vi "Test Time Entry Month Files.vi"(8 "error in (no error)":errorcluster, 10 "Work Folder":path, 11 "Test Data Folder":path) -> (0 "error out":errorcluster, 2 "Report":string, 3 "Passed":bool)   [LabVIEW 2024]
doc: "Saves two entries with Time Entry Store-INI: one that starts on 30 Sep 2025 22:30 UTC (already 1 October in Central European time, and saved while today is in October) and one that runs from 31 Oct 23:30 UTC into November. The month file is chosen by the UTC Start Time, so the first must land in 2025-09.ini only and the second in 2025-10.ini only.\n\nInputs: Test Data Folder holds the source copies (Samples, v1); each run works in a new case folder under Work Folder. Passed is TRUE when every check passed and no error occurred; Report lists every check.\n\nGenerated by: Claude"
uses:
  Storage/Project Store-INI/Project Store-INI.lvclass
  Storage/Time Entry Store-INI/Time Entry Store-INI.lvclass
  Utilities/Time Management/Time Management.lvlib
  Storage/Time Entry Store/Time Entry Store.lvclass
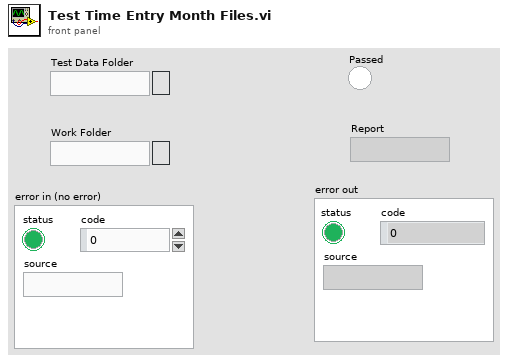
[diagram p1: front panel]
types:
  T1 = cluster{"c6018":string, "c6019":string, "c6020":string, "Timestamp":timestamp, "Timestamp":timestamp, "c6021":string}
  T2 = typedef "Time Entry.ctl" = cluster{"ID":string, "Project ID":string, "Task ID":string, "Start Time":timestamp, "End Time":timestamp, "Description":string}
  T3 = cluster{"c6030":string, "c6031":string, "c6032":string, "Timestamp":timestamp, "Timestamp":timestamp, "c6033":string}
  T4 = typedef "Time Entry List.ctl" = T2[]
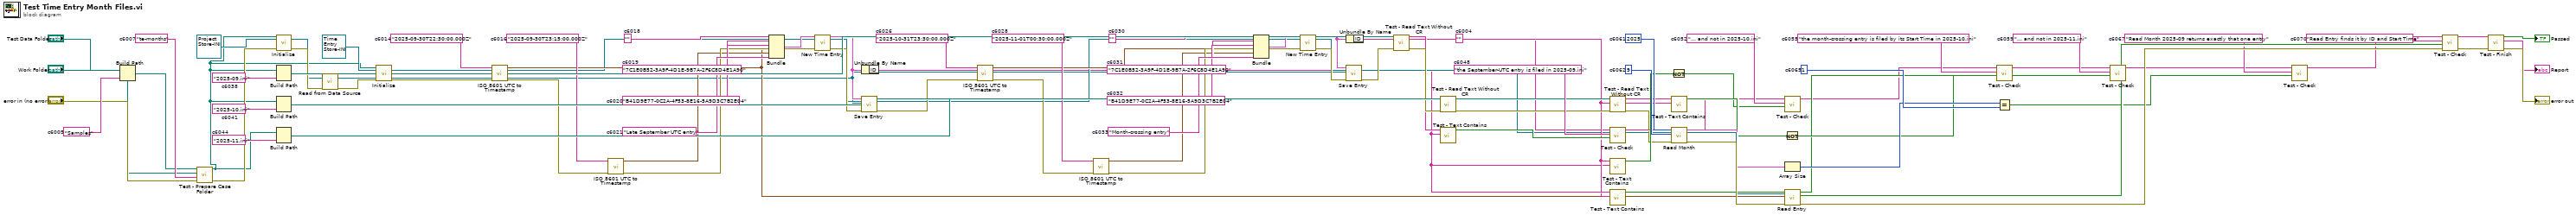
[diagram p0: block diagram]
diagram:
  w90 = "Read Entry finds it by ID and Start Time"  # c6070
  w86 = "Read Month 2025-09 returns exactly that one entry"  # c6067
  w84 = 1  # c6065
  w79 = 9  # c6062
  w78 = 2025  # c6061
  w76 = "... and not in 2025-11.ini"  # c6059
  w72 = "the month-crossing entry is filed by its Start Time in 2025-10.ini"  # c6055
  w69 = "... and not in 2025-10.ini"  # c6052
  w65 = "the September-UTC entry is filed in 2025-09.ini"  # c6048
  w60 = "2025-11.ini"  # c6044
  w56 = "2025-10.ini"  # c6041
  w52 = "2025-09.ini"  # c6038
  w44 = "Month-crossing entry"  # c6033
  w43 = "B41D9E77-0C2A-4F53-8E16-5A9D3C7B2E04"  # c6032
  w42 = "7C1E0B52-3A9F-4D1E-9B7A-2F6C8D4E1A90"  # c6031
  w41 = ""  # c6030
  w38 = "2025-11-01T00:30:00.000Z"  # c6028
  w35 = "2025-10-31T23:30:00.000Z"  # c6026
  w27 = "Late September UTC entry"  # c6021
  w26 = "B41D9E77-0C2A-4F53-8E16-5A9D3C7B2E04"  # c6020
  w25 = "7C1E0B52-3A9F-4D1E-9B7A-2F6C8D4E1A90"  # c6019
  w24 = ""  # c6018
  w21 = "2025-09-30T23:15:00.000Z"  # c6016
  w18 = "2025-09-30T22:30:00.000Z"  # c6014
  w7 = "te-months"  # c6007
  w5 = "Samples"  # c6005
  w4 = ""  # c6004
  n1 = Build Path(base path="Test Data Folder", name or relative path=w5) -> (appended path=w6:path)
  n2 = call "Test - Prepare Case Folder.vi"("error in (no error)"="error in (no error)", "Case Name"=w7, "Work Folder"="Work Folder", "Source Folder"=w6) -> ("error out"=w9:errorcluster, "Case Folder"=w8:path)  [unwired: 6 in]
  n3 = call-dynamic "Initialize.vi"("Project Store in"=refnum<class "Project Store-INI.lvclass"> refnum ("Project Store-INI"), "error in (no error)"=w9, "Data Folder"=w8) -> ("error out"=w12:errorcluster, "Project Store out"=w11:refnum<class "Project Store-INI.lvclass">)  [unwired: 7 in]
  n4 = Build Path(base path=w8, name or relative path=w52) -> (appended path=w53:path)
  n5 = Build Path(base path=w8, name or relative path=w56) -> (appended path=w57:path)
  n6 = Build Path(base path=w8, name or relative path=w60) -> (appended path=w61:path)
  n7 = call-dynamic "Read from Data Source.vi"("Project Store in"=w11, "error in (no error)"=w12) -> ("error out"=w14:errorcluster, "Project Store out"=w13:refnum<class "Project Store-INI.lvclass">)  [unwired: 8 in]
  n8 = call-dynamic "Initialize.vi"("Time Entry Store in"=refnum<class "Time Entry Store-INI.lvclass"> refnum ("Time Entry Store-INI"), "error in (no error)"=w14, "Data Folder"=w8) -> ("error out"=w17:errorcluster, "Time Entry Store out"=w16:refnum<class "Time Entry Store-INI.lvclass">)  [unwired: 7 in]
  n9 = call "ISO 8601 UTC to Timestamp.vi"("error in (no error)"=w17, "ISO 8601 UTC"=w18) -> ("error out"=w20:errorcluster, "Timestamp"=w19:timestamp)  [unwired: 8 in]
  n10 = call "ISO 8601 UTC to Timestamp.vi"("error in (no error)"=w20, "ISO 8601 UTC"=w21) -> ("error out"=w23:errorcluster, "Timestamp"=w22:timestamp)  [unwired: 8 in]
  n11 = Bundle("c6018"=w24, "c6019"=w25, "c6020"=w26, "Timestamp"=w19, "Timestamp"=w22, "c6021"=w27) -> (w28:T1)  [unwired: 1 in]
  n12 = call "New Time Entry.vi"("Time Entry Store in"=w16, "error in (no error)"=w23, "Time Entry"=w28) -> ("error out"=w31:errorcluster, "New Time Entry"=w29:T2, "Time Entry Store out"=w30:refnum<class "Time Entry Store-INI.lvclass">)  [unwired: 6 in]
  n13 = Unbundle By Name(w29) -> ("ID"=w32:string)
  n14 = call-dynamic "Save Entry.vi"("Time Entry Store in"=w30, "error in (no error)"=w31, "Project Store"=w13, "Time Entry"=w29) -> ("error out"=w34:errorcluster, "Time Entry Store out"=w33:refnum<class "Time Entry Store-INI.lvclass">)  [unwired: 6 in]
  n15 = call "ISO 8601 UTC to Timestamp.vi"("error in (no error)"=w34, "ISO 8601 UTC"=w35) -> ("error out"=w37:errorcluster, "Timestamp"=w36:timestamp)  [unwired: 8 in]
  n16 = call "ISO 8601 UTC to Timestamp.vi"("error in (no error)"=w37, "ISO 8601 UTC"=w38) -> ("error out"=w40:errorcluster, "Timestamp"=w39:timestamp)  [unwired: 8 in]
  n17 = Bundle("c6030"=w41, "c6031"=w42, "c6032"=w43, "Timestamp"=w36, "Timestamp"=w39, "c6033"=w44) -> (w45:T3)  [unwired: 1 in]
  n18 = call "New Time Entry.vi"("Time Entry Store in"=w33, "error in (no error)"=w40, "Time Entry"=w45) -> ("error out"=w48:errorcluster, "New Time Entry"=w46:T2, "Time Entry Store out"=w47:refnum<class "Time Entry Store-INI.lvclass">)  [unwired: 6 in]
  n19 = Unbundle By Name(w46) -> ("ID"=w49:string)
  n20 = call-dynamic "Save Entry.vi"("Time Entry Store in"=w47, "error in (no error)"=w48, "Project Store"=w13, "Time Entry"=w46) -> ("error out"=w51:errorcluster, "Time Entry Store out"=w50:refnum<class "Time Entry Store-INI.lvclass">)  [unwired: 6 in]
  n21 = call "Test - Read Text Without CR.vi"("error in (no error)"=w51, "File"=w53) -> ("error out"=w55:errorcluster, "Text"=w54:string)  [unwired: 8 in]
  n22 = call "Test - Read Text Without CR.vi"("error in (no error)"=w55, "File"=w57) -> ("error out"=w59:errorcluster, "Text"=w58:string)  [unwired: 8 in]
  n23 = call "Test - Text Contains.vi"("Search Text"=w32, "Text"=w54) -> ("Contains?"=w64:bool)  [unwired: 8 in, 1 out]
  n24 = call "Test - Read Text Without CR.vi"("error in (no error)"=w59, "File"=w61) -> ("error out"=w63:errorcluster, "Text"=w62:string)  [unwired: 8 in]
  n25 = call "Test - Check.vi"("Condition"=w64, "Check Name"=w65, "Report in"=w4) -> ("Report out"=w66:string)  [unwired: 7 in, 1 out]
  n26 = call "Test - Text Contains.vi"("Search Text"=w32, "Text"=w58) -> ("Contains?"=w67:bool)  [unwired: 8 in, 1 out]
  n27 = call "Test - Text Contains.vi"("Search Text"=w49, "Text"=w58) -> ("Contains?"=w71:bool)  [unwired: 8 in, 1 out]
  n28 = Not(x=w67) -> (.not. x?=w68:bool)
  n29 = call "Test - Text Contains.vi"("Search Text"=w49, "Text"=w62) -> ("Contains?"=w74:bool)  [unwired: 8 in, 1 out]
  n30 = call-dynamic "Read Month.vi"("Time Entry Store in"=w50, "error in (no error)"=w63, "Month"=w79, "Year"=w78) -> ("error out"=w82:errorcluster, "Time Entries"=w80:T4, "Time Entry Store out"=w81:refnum<class "Time Entry Store-INI.lvclass">)  [unwired: 5 in]
  n31 = call "Test - Check.vi"("Condition"=w68, "Check Name"=w69, "Report in"=w66) -> ("Report out"=w70:string)  [unwired: 7 in, 1 out]
  n32 = Not(x=w74) -> (.not. x?=w75:bool)
  n33 = Array Size(array=w80) -> (size(s)=w83:i32)
  n34 = call-dynamic "Read Entry.vi"("Time Entry Store in"=w81, "error in (no error)"=w82, "Start Time"=w19, "ID"=w32) -> ("error out"=w89:errorcluster, "found?"=w88:bool)  [unwired: 4 in, 2 out]
  n35 = call "Test - Check.vi"("Condition"=w71, "Check Name"=w72, "Report in"=w70) -> ("Report out"=w73:string)  [unwired: 7 in, 1 out]
  n36 = Equal?(x=w83, y=w84) -> (x = y?=w85:bool)
  n37 = call "Test - Check.vi"("Condition"=w75, "Check Name"=w76, "Report in"=w73) -> ("Report out"=w77:string)  [unwired: 7 in, 1 out]
  n38 = call "Test - Check.vi"("Condition"=w85, "Check Name"=w86, "Report in"=w77) -> ("Report out"=w87:string)  [unwired: 7 in, 1 out]
  n39 = call "Test - Check.vi"("Condition"=w88, "Check Name"=w90, "Report in"=w87) -> ("Report out"=w91:string)  [unwired: 7 in, 1 out]
  n40 = call "Test - Finish.vi"("error in (no error)"=w89, "Report"=w91) -> ("error out"=→"error out":errorcluster, "Report out"=→"Report":string, "Passed"=→"Passed":bool)  [unwired: 7 in]
